vi "To and  From String Array.vi"() -> (0 "error out":errorcluster, 3 "Pass":bool)   [LabVIEW 2015, in "DAQmx Module Tests.lvlib"]
uses:
  DAQmx Module Tests.lvlib
  <vilib>/NI/Tag Bus Module Framework/channel/channel classification.ctl
  <vilib>/NI/Tag Bus/tag/Data Type.ctl
  module/configuration/Daqmx Module configuration.lvclass/Daqmx Module configuration.ctl
  <vilib>/NI/Tag Bus/tag/tag descriptor.lvclass/tag descriptor.ctl
  <vilib>/NI/Tag Bus Module Framework/channel/TBM channel.lvclass/TBM channel.ctl
  <vilib>/NI/Tag Bus Module Framework/channel/TBM channel.lvclass
  module/configuration/Daqmx Module configuration.lvclass
  <vilib>/NI/Tag Bus/tag/tag descriptor.lvclass
panel:
  out "x = y?":T1(array[cluster])
  out "data type 2":T2
  out "data type":T2
  in  "index":i32
  out "name 2":string
  out "name":string
  out "channel classification 2":T3
  out "channel classification":T3
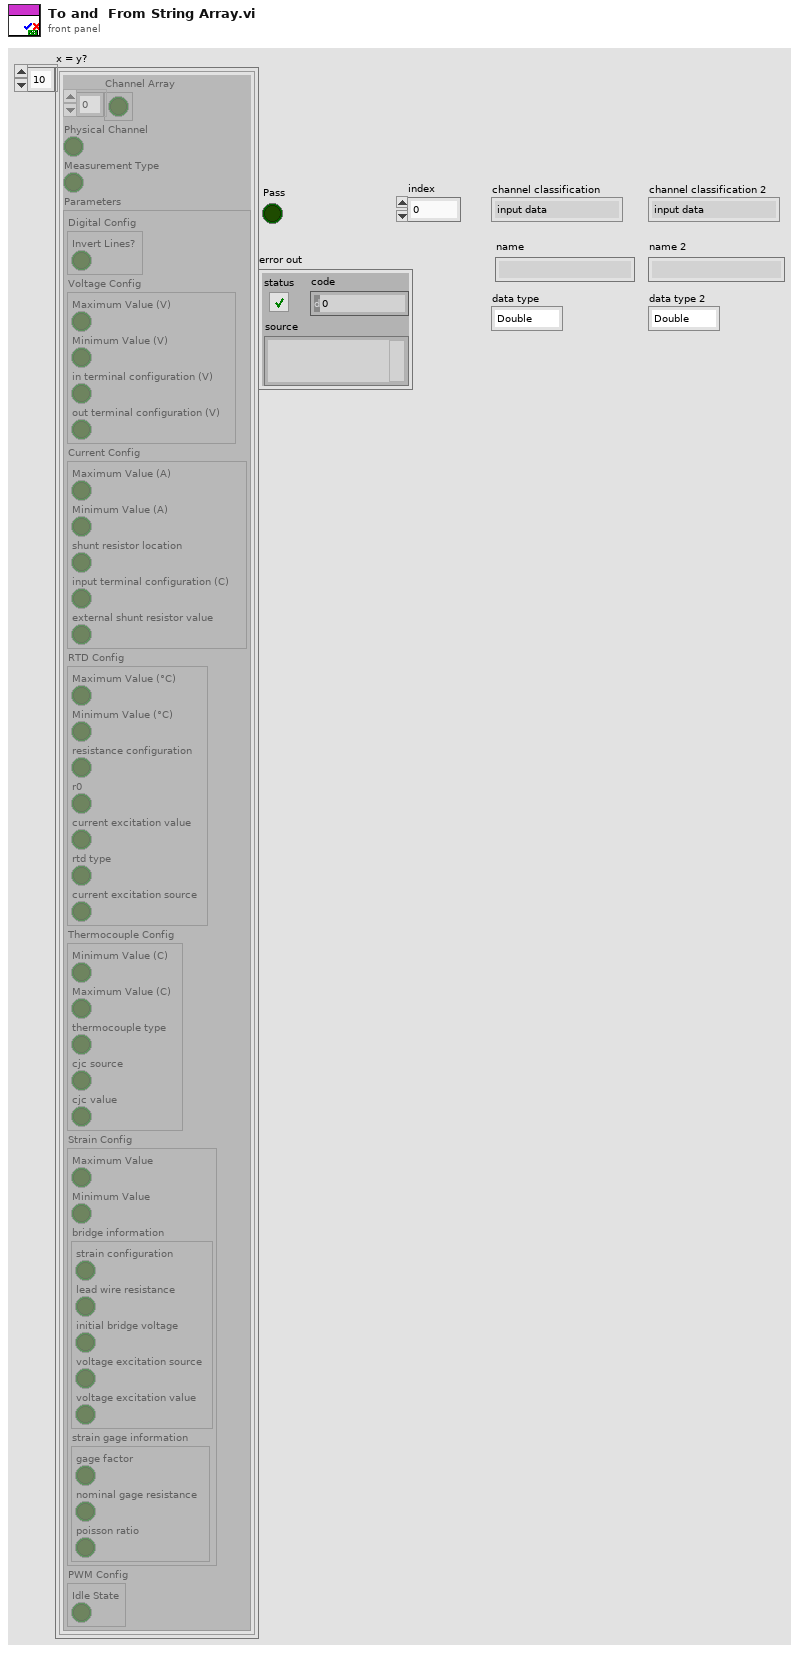
[diagram p1: front panel]
types:
  T1 = cluster{"Channel Array":bool[], "Physical Channel":bool, "Measurement Type":bool, "Parameters":cluster{"Digital Config":cluster{"Invert Lines?":bool}, "Voltage Config":cluster{"Maximum Value (V)":bool, "Minimum Value (V)":bool, "in terminal configuration (V)":bool, "out terminal configuration (V)":bool}, "Current Config":cluster{"Maximum Value (A)":bool, "Minimum Value (A)":bool, "shunt resistor location":bool, "input terminal configuration (C)":bool, "external shunt resistor value":bool}, "RTD Config":cluster{"Maximum Value (°C)":bool, "Minimum Value (°C)":bool, "resistance configuration":bool, "r0":bool, "current excitation value":bool, "rtd type":bool, "current excitation source":bool}, "Thermocouple Config":cluster{"Minimum Value (C)":bool, "Maximum Value (C)":bool, "thermocouple type":bool, "cjc source":bool, "cjc value":bool}, "Strain Config":cluster{"Maximum Value":bool, "Minimum Value":bool, "bridge information":cluster{"strain configuration":bool, "lead wire resistance":bool, "initial bridge voltage":bool, "voltage excitation source":bool, "voltage excitation value":bool}, "strain gage information":cluster{"gage factor":bool, "nominal gage resistance":bool, "poisson ratio":bool}}, "PWM Config":cluster{"Idle State":bool}}}[]
  T2 = typedef "tag bus.lvlib/tag descriptor.lvclass/Data Type.ctl" = enum16{"Double", "Single", "I64", "I32", "I16", "I8", "U64", "U32", "U16", "U8", "Boolean", "String", "Array of Double", "Array of Single", "Array of I64", "Array of I32", "Array of I16", "Array of I8", "Array of U64", "Array of U32", "Array of U16", "Array of U8", "Array of Boolean", "Array of String"}
  T3 = typedef "TBM channel.lvclass/channel classification.ctl" = enum16{"input data", "output data", "processing parameter", "processing result"}
  T4 = typedef "DAQmx Module Configuration.lvclass/Line.ctl" = cluster{"Channel Array":refnum<class "TBM channel.lvclass">[], "Physical Channel":string, "Measurement Type":T5, "Parameters":T6}
  T5 = typedef "DAQmx Module Configuration.lvclass/Measurement Type.ctl" = enum16{"Digital Input", "Digital Output", "Voltage Input", "Voltage Output", "Current Input", "Current Output", "RTD", "Thermocouple", "Strain", "PWM"}
  T6 = typedef "DAQmx Module Configuration.lvclass/Parameters.ctl" = cluster{"Digital Config":cluster{"Invert Lines?":bool}, "Voltage Config":cluster{"Maximum Value (V)":dbl, "Minimum Value (V)":dbl, "in terminal configuration (V)":i32, "out terminal configuration (V)":i32}, "Current Config":cluster{"Maximum Value (A)":dbl, "Minimum Value (A)":dbl, "shunt resistor location":i32, "input terminal configuration (C)":i32, "external shunt resistor value":dbl}, "RTD Config":cluster{"Maximum Value (°C)":dbl, "Minimum Value (°C)":dbl, "resistance configuration":i32, "r0":dbl, "current excitation value":dbl, "rtd type":i32, "current excitation source":i32}, "Thermocouple Config":cluster{"Minimum Value (C)":dbl, "Maximum Value (C)":dbl, "thermocouple type":i32, "cjc source":i32, "cjc value":dbl}, "Strain Config":cluster{"Maximum Value":dbl, "Minimum Value":dbl, "bridge information":cluster{"strain configuration":i32, "lead wire resistance":dbl, "initial bridge voltage":dbl, "voltage excitation source":i32, "voltage excitation value":dbl}, "strain gage information":cluster{"gage factor":dbl, "nominal gage resistance":dbl, "poisson ratio":dbl}}, "PWM Config":cluster{"Idle State":bool}}
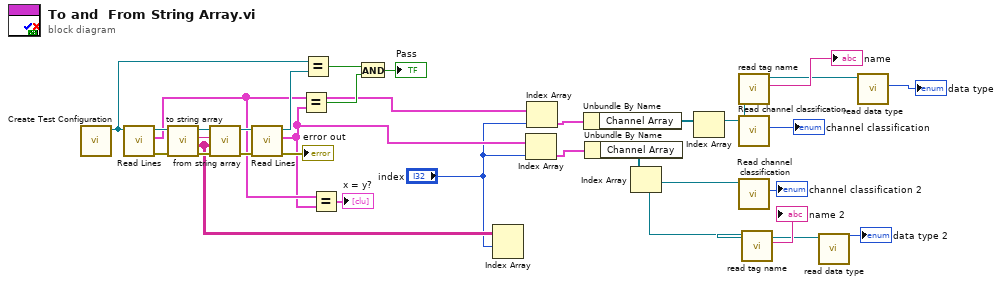
[diagram p0: block diagram]
diagram:
  n1 = call "Create Test Configuration.vi"() -> ("Module Configuration"=w24:refnum<class "Daqmx Module configuration.lvclass">)  [unwired: 7 in, 4 out]
  n2 = call "Read Lines.vi"("Daqmx Module configuration in"=w24) -> ("error out"=w28:errorcluster, "Lines"=w19:T4[], "Daqmx Module configuration out"=w30:refnum<class "Daqmx Module configuration.lvclass">)  [unwired: 8 in]
  n3 = call-dynamic "to string array.vi"("error in (no error)"=w28, "module configuration in"=w30) -> ("error out"=w27:errorcluster, "Array"=w5:string[][], "version"=w32:string, "module configuration out"=w31:refnum<class "Daqmx Module configuration.lvclass">)  [unwired: 6 in]
  n4 = call-dynamic "from string array.vi"("error in (no error)"=w27, "String Array"=w5, "version"=w32, "module configuration in"=w31) -> ("error out"=w26:errorcluster, "module configuration out"=w29:refnum<class "Daqmx Module configuration.lvclass">)  [unwired: 6 in]
  n5 = call "Read Lines.vi"("error in (no error)"=w26, "Daqmx Module configuration in"=w29) -> ("error out"=→"error out":errorcluster, "Lines"=w18:T4[], "Daqmx Module configuration out"=w23:refnum<class "Daqmx Module configuration.lvclass">)  [unwired: 7 in]
  n6 = Equal?(x=w19, y=w18) -> (x = y?=w21:bool)
  n7 = Equal?(x=w24, y=w23) -> (x = y?=w22:bool)
  n8 = Equal?(x=w19, y=w18) -> (x = y?=→"x = y?":T1)
  n9 = And(x=w22, y=w21) -> (x .and. y?=→"Pass":bool)
  n10 = Index Array(array=w5, index (row)="index") -> ()  [unwired: 1 in, 1 out]
  n11 = Index Array(array=w18, index="index") -> (element=w16:T4)
  n12 = Index Array(array=w19, index="index") -> (element=w17:T4)
  n13 = Unbundle By Name(w17) -> ("Channel Array"=w13:refnum<class "TBM channel.lvclass">[])
  n14 = Unbundle By Name(w16) -> ("Channel Array"=w12:refnum<class "TBM channel.lvclass">[])
  n15 = Index Array(array=w12) -> (element=w2:refnum<class "TBM channel.lvclass">)  [unwired: 1 in]
  n16 = Index Array(array=w13) -> (element=w3:refnum<class "TBM channel.lvclass">)  [unwired: 1 in]
  n17 = call <vilib>:"read tag name.vi"("system tag in"=w3) -> ("name"=→"name":string, "system tag out"=w9:refnum<class "TBM channel.lvclass">)  [unwired: 8 in, 1 out]
  n18 = call <vilib>:"Read channel classification.vi"("channel in"=w3) -> ("channel classification"=→"channel classification":T3)  [unwired: 8 in, 2 out]
  n19 = call <vilib>:"Read channel classification.vi"("channel in"=w2) -> ("channel classification"=→"channel classification 2":T3)  [unwired: 8 in, 2 out]
  n20 = call <vilib>:"read tag name.vi"("system tag in"=w2) -> ("name"=→"name 2":string, "system tag out"=w8:refnum<class "TBM channel.lvclass">)  [unwired: 8 in, 1 out]
  n21 = call <vilib>:"read data type.vi"("system tag in"=w8) -> ("data type"=→"data type 2":T2)  [unwired: 8 in, 2 out]
  n22 = call <vilib>:"read data type.vi"("system tag in"=w9) -> ("data type"=→"data type":T2)  [unwired: 8 in, 2 out]
